vi "LogViewer.vi"(7 "Current Module(\"\" to generate an ID)":string="logViewer") -> ()   [LabVIEW 2017, in "DebugConsole.lvlib"]
uses:
  DebugConsole.lvlib
  Utility/_support/Periodic String Filter Level.ctl
  _BroadcastDef.ctl
  Utility/Periodic String Filter Setting.ctl
  _Shared/Change Speed Counter.vi
  _Shared/Rising Edge.vi
  _Shared/Debounced Signal.vi
  _csmlite/_PassAllowedMessage - MsgList.vi
  Communicable State Machine.lvlib
  _Shared/CSM Shared.lvlib
  _Support/csm-tool-support.lvlib
  _csmHelper/API with lvcsm Support/CSM-Helper API with lvcsm Support.lvlib
  addons/Logger/CSM File Logger.lvlib
  _ui/csm-ui-support.lvlib
  _csmlite/_csmlite.lvlib
panel:
  out "Error(#)":i64 caption="Error(#):"
  in  "Record.Stop":bool
  in  "Record.Start":bool
  in  "Clear":bool
  in  "BackTop":bool
  in  "Toolbar.History Length(char)":i32=50000 caption="History(char)" min=1000 max=100000000 step=1
  in  "Peroid Logs":bool
  in  "Tab":T1(tab)
  out "State History":string
  out "Error History":string
  out "Userlog History":string
  out "Global Filters":string
  out "LogInQ":i32 caption="LogInQ:"
  out "log handling Speed(#/s)":dbl caption="log handling Speed(#/s):"
  out "LogInQ change(#/s)":dbl caption="LogInQ change(#/s):"
  out "Level":T2 caption="Level:"
  in  "Stop":bool
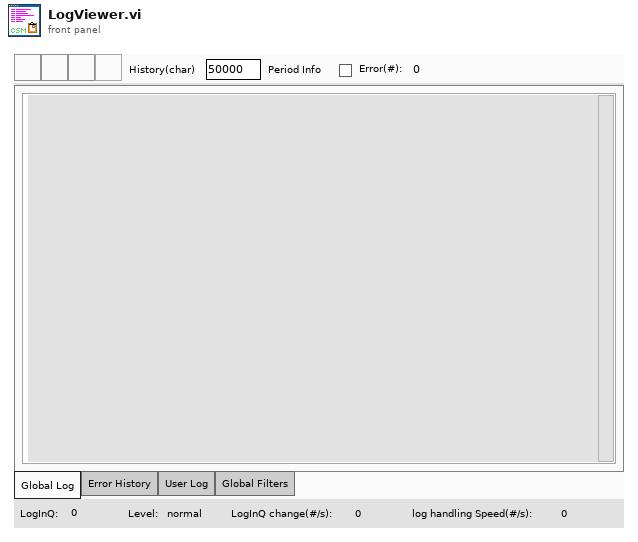
[diagram p1: front panel]
types:
  T1 = enum32{"Global Log", "Error History", "User Log", "Global Filters"}
  T2 = typedef "Communicable State Machine.lvlib/Periodic String Filter Level.ctl" = enum16{"normal", "L1", "L2", "L3", "L4"}
  T3 = typedef "DebugConsole.lvlib/_BroadcastDef.ctl" = enum16{"<no action>", "Macro: Exit", "CSM: Module List Changed", "CSM: Scripts Changed", "CSM: Registration Changed", "CSM: Module Selected", "CSM: Message Excuted", "CSM: Broadcast Excuted", "CSM: Registration Action Excuted", "UI: Try to Change Command"}
  T4 = typedef "Communicable State Machine.lvlib/Periodic String Filter Setting.ctl" = cluster{"threashold(#/s)":dbl, "Check Peroid(s)":dbl}
  T5 = typedef "Communicable State Machine.lvlib/_CSM_GlobalLog_MSG.ctl" = cluster{"Name (\"\" to Use UUID)":string, "Current State":string, "Arguments":string, "Source Message":T6, "Source Module":string, "Complete(T)/Start(F)":bool, "LogType":T7, "Time Stamp":timestamp}
  T6 = typedef "Communicable State Machine.lvlib/_CSM_Response Source Message.ctl" = cluster{"‘State":string, "’Arguments":string, "’Error":errorcluster}
  T7 = typedef "Communicable State Machine.lvlib/_CSM_GlobalLog_MSG_TYPE.ctl" = enum16{"User Log", "State Change", "Status", "Interrupt", "Register", "Unregister", "Error Log", "Module Created", "Module Destroyed", "Async Message", "No-Rep Async Message", "Sync Message"}
  T8 = enum32{"Invalid", "Standard", "Closed", "Hidden", "Minimized", "Maximized"}
  T9 = enum32{"invalid app kind", "Development System", "Run Time System", "Student Edition", "Embedded LabVIEW", "Evaluation", "Custom"}
  T10 = typedef "LVPoint32TypeDef.ctl" = cluster{"Horizontal":i32, "Vertical":i32}
  T11 = cluster{"Shift":bool, "Ctrl":bool, "Alt":bool, "Cmd":bool, "Opt":bool}
  T12 = cluster{"Core":cluster{"Current VI Reference":refnum<vi>, "Close Panel on Exit?":bool}, "Toolbar.Advance":refnum<vi>[], "LoggerWatchDogQueue":refnum<queue>, "LogFile":path}
  T13 = cluster{"Current VI Reference":refnum<vi>, "Close Panel on Exit?":bool}
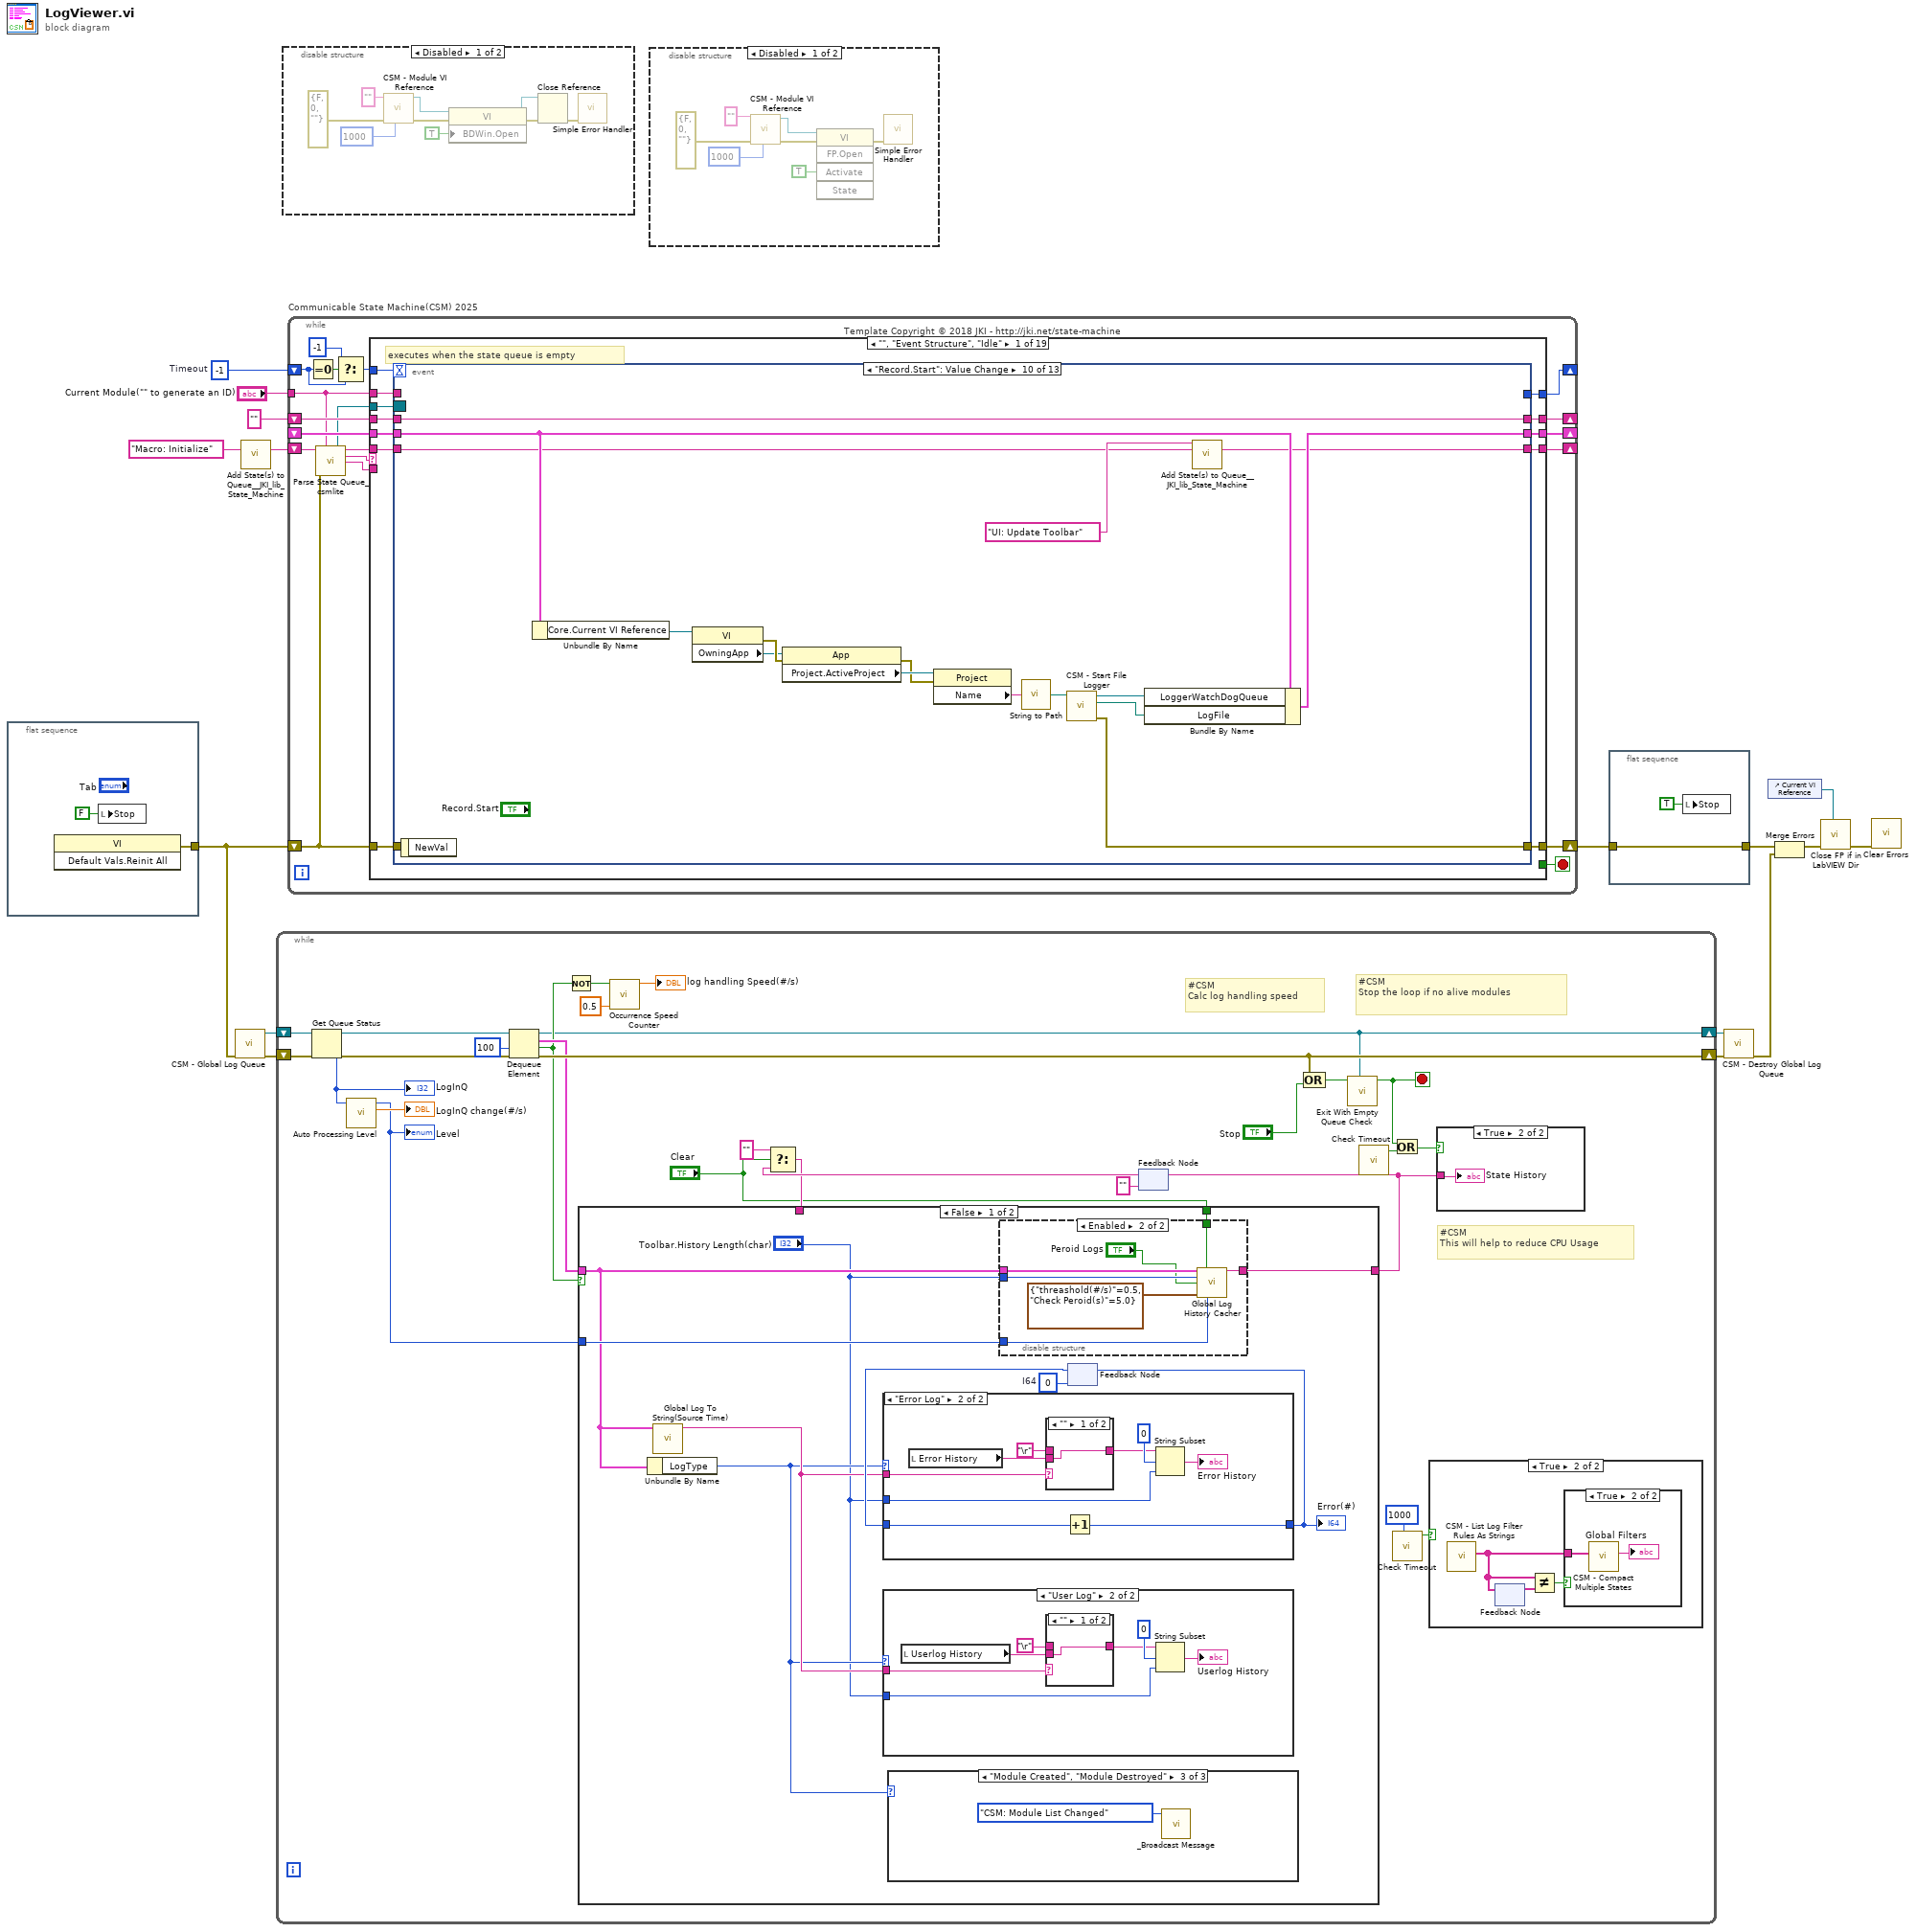
[diagram p0: block diagram]
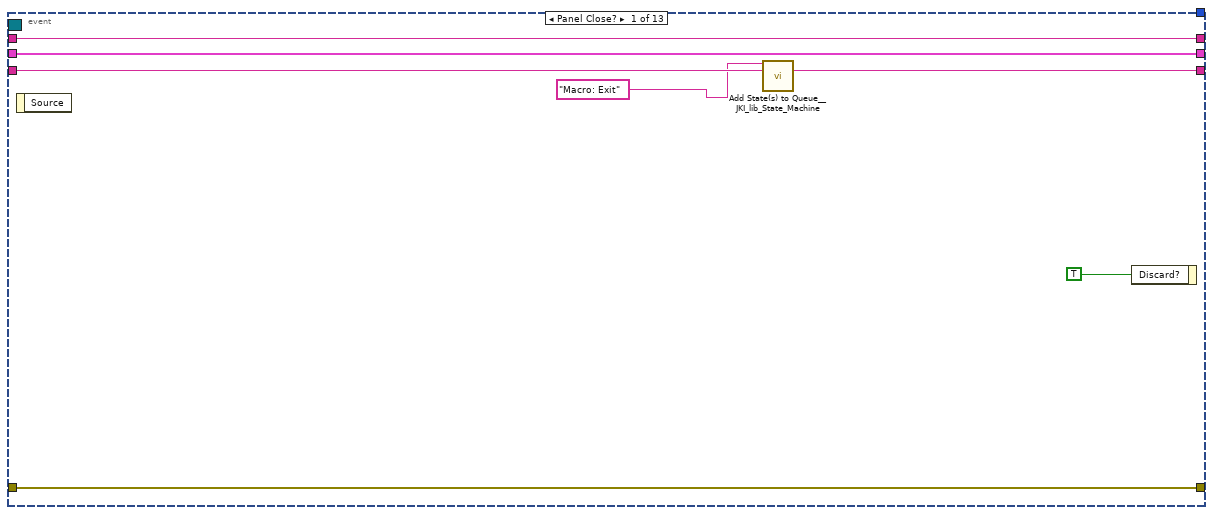
[diagram p4: hidden frame]
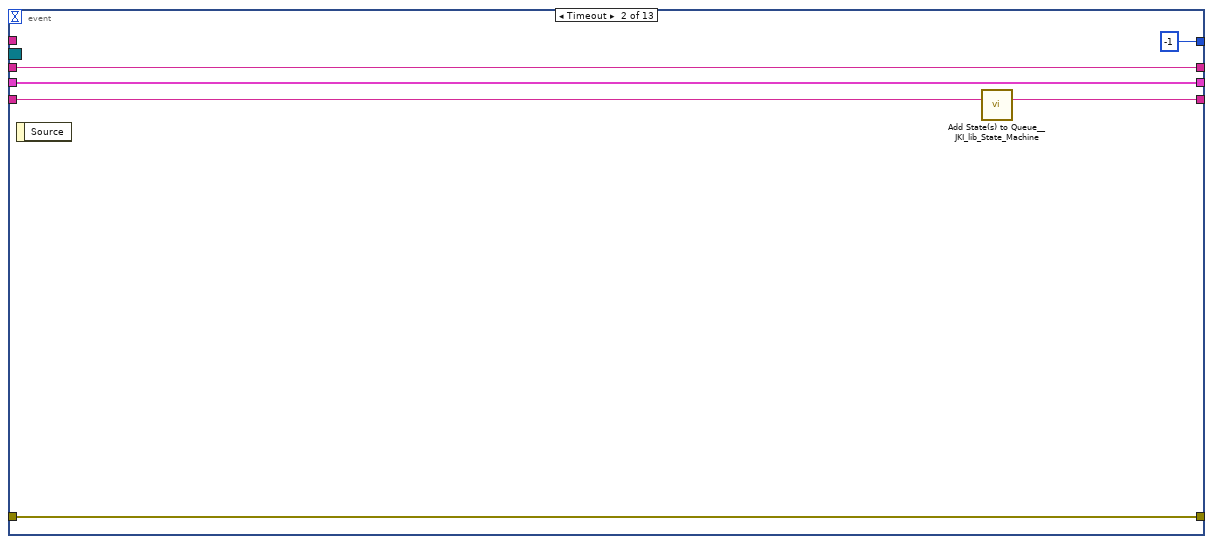
[diagram p5: hidden frame]
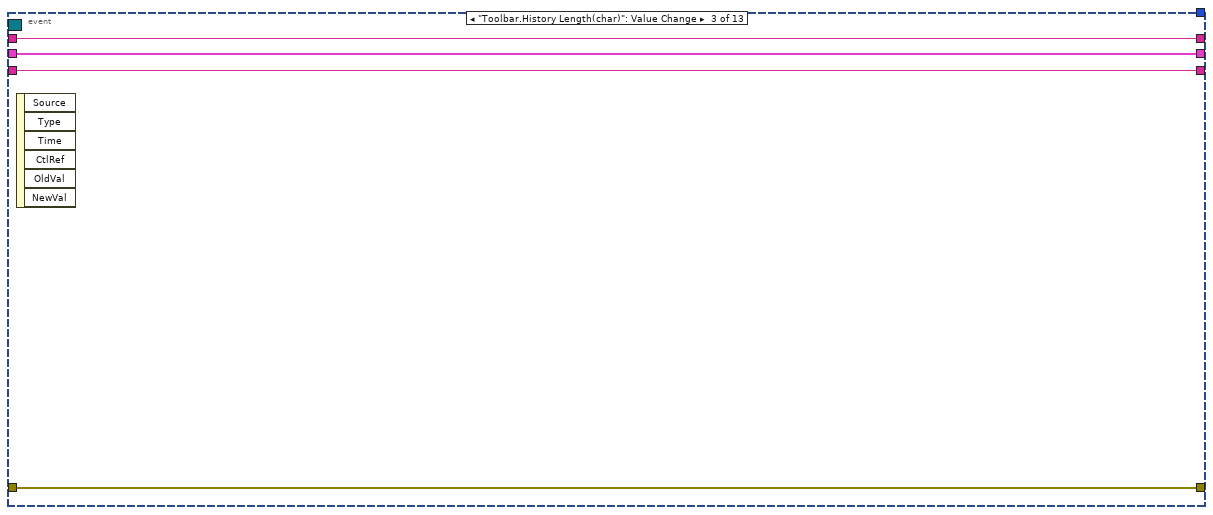
[diagram p6: hidden frame]
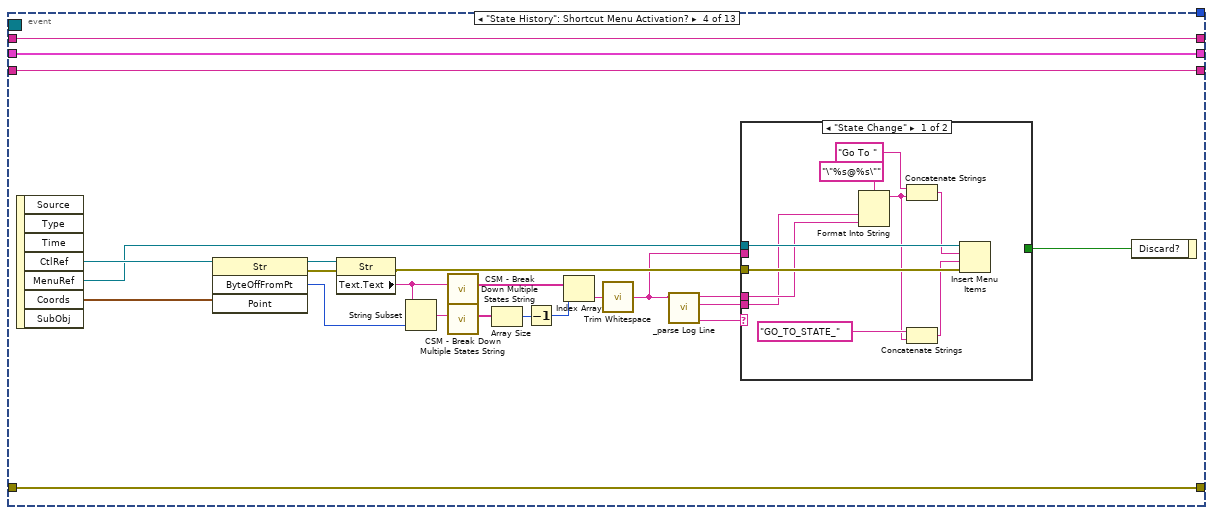
[diagram p7: hidden frame]
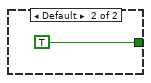
[diagram p8: hidden frame]
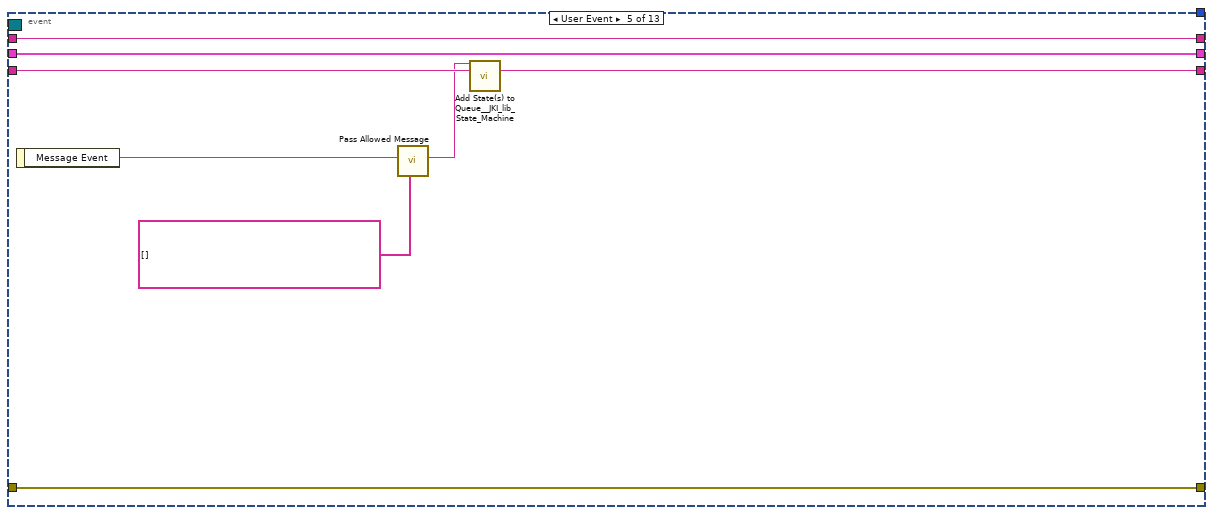
[diagram p9: hidden frame]
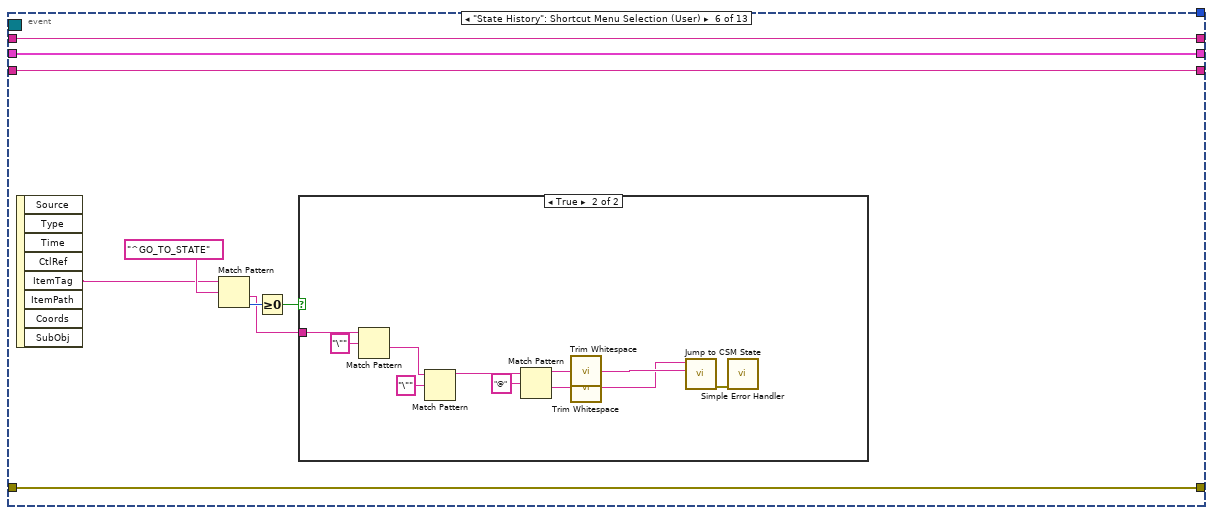
[diagram p10: hidden frame]
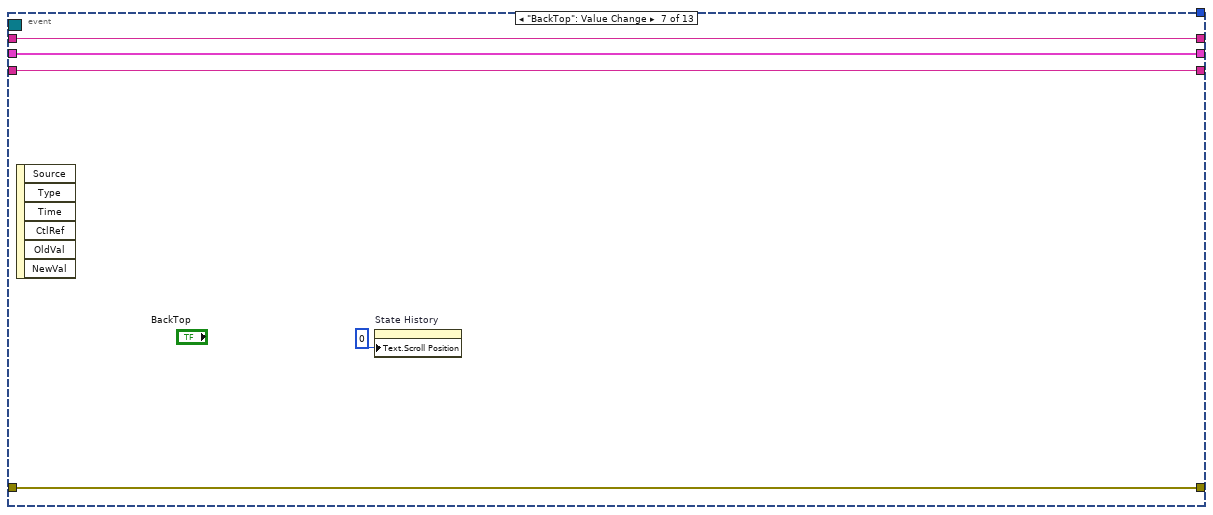
[diagram p12: hidden frame]
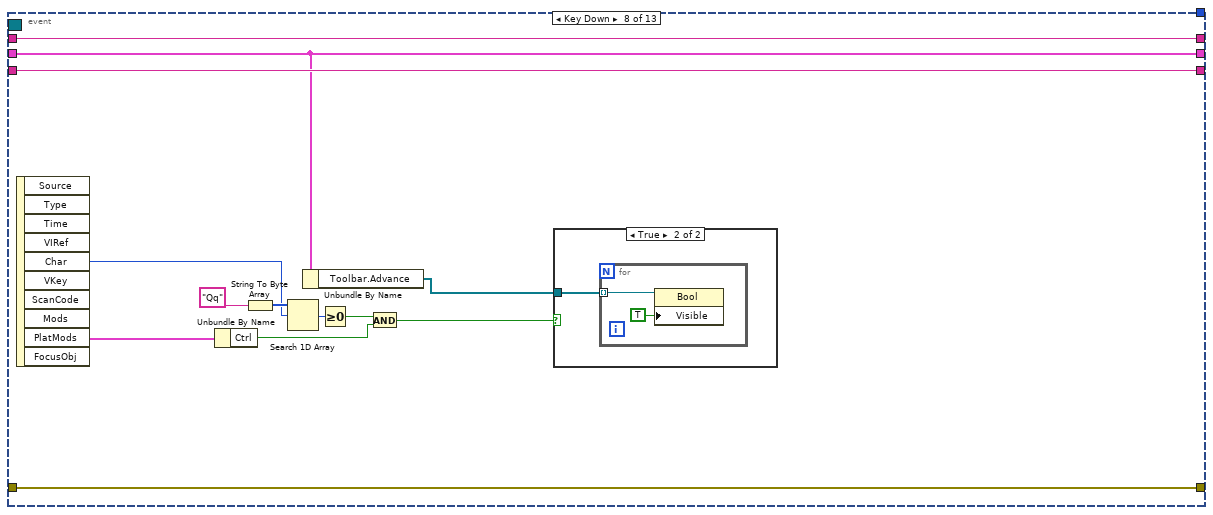
[diagram p13: hidden frame]
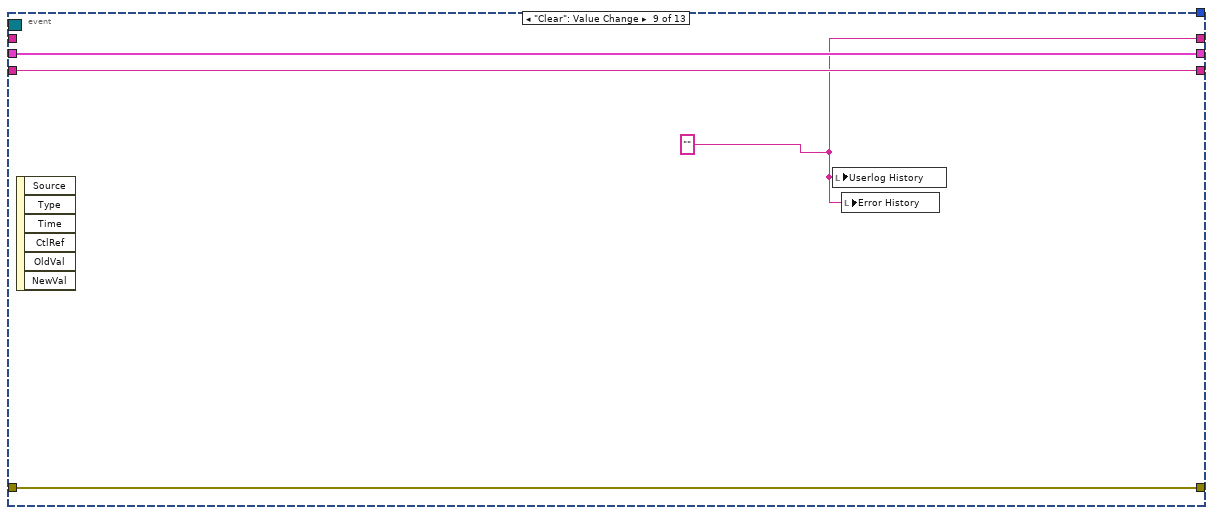
[diagram p15: hidden frame]
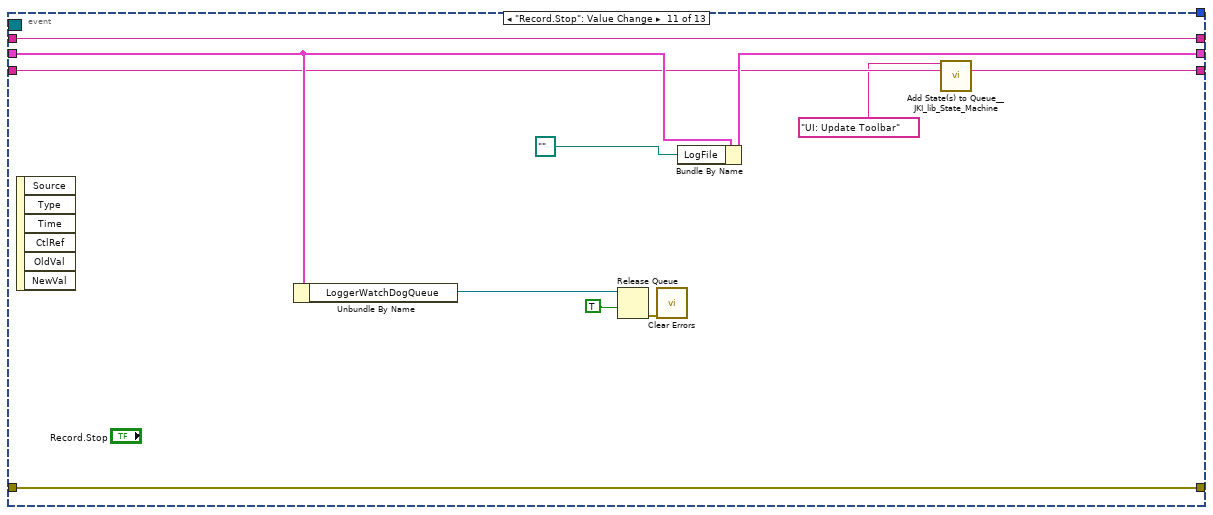
[diagram p16: hidden frame]
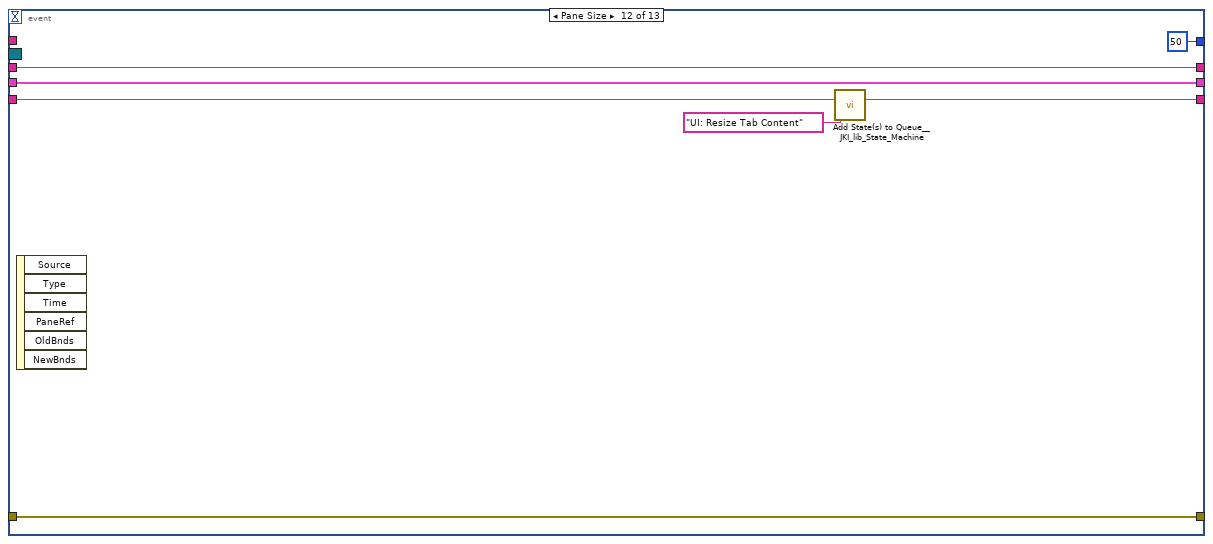
[diagram p17: hidden frame]
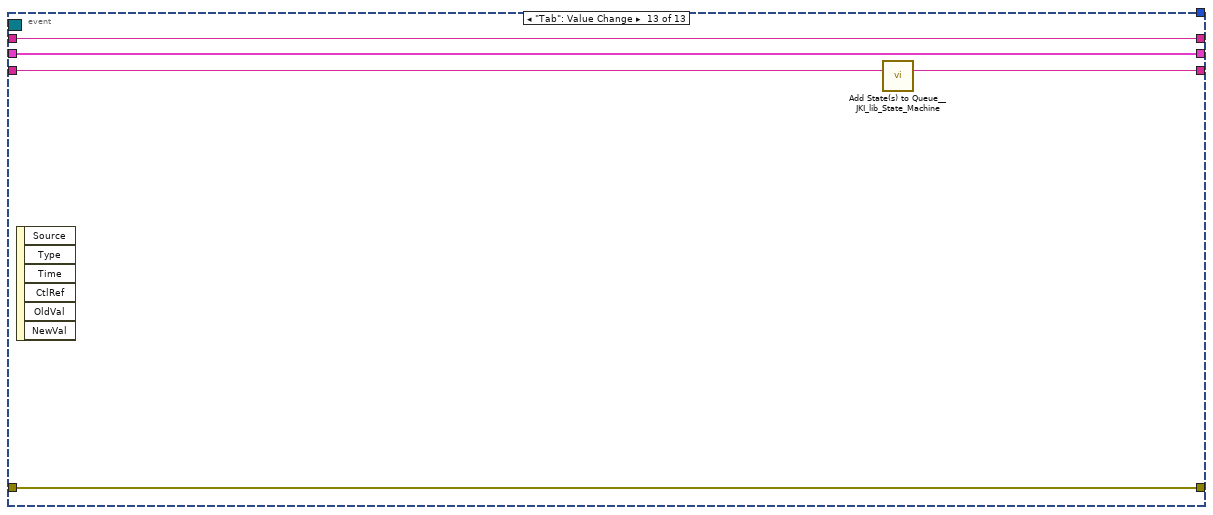
[diagram p18: hidden frame]
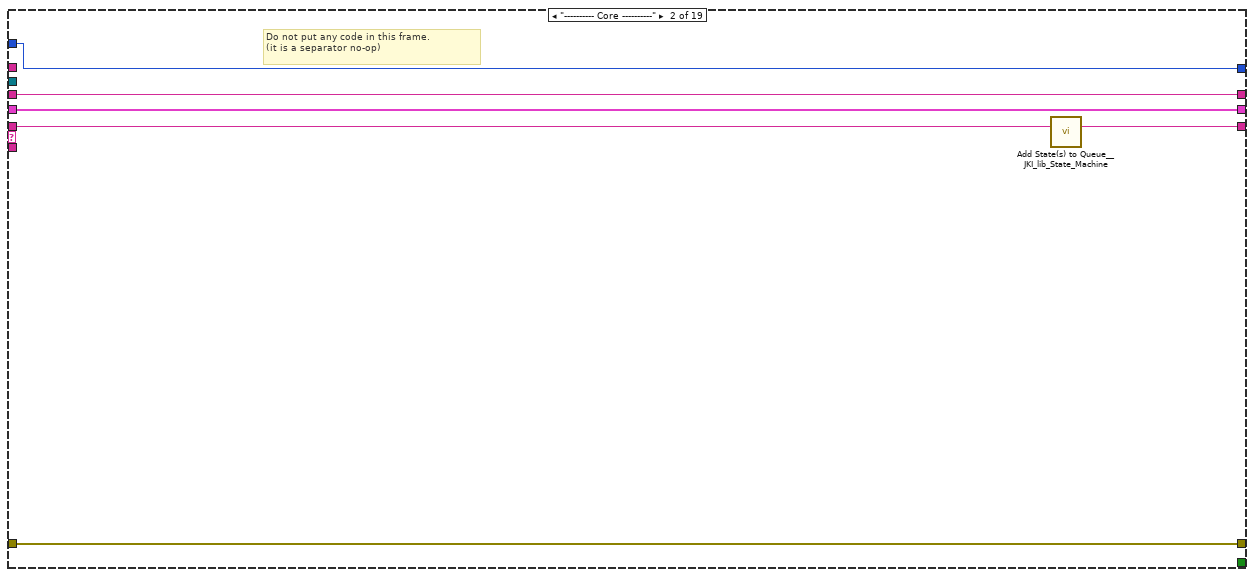
[diagram p19: hidden frame]
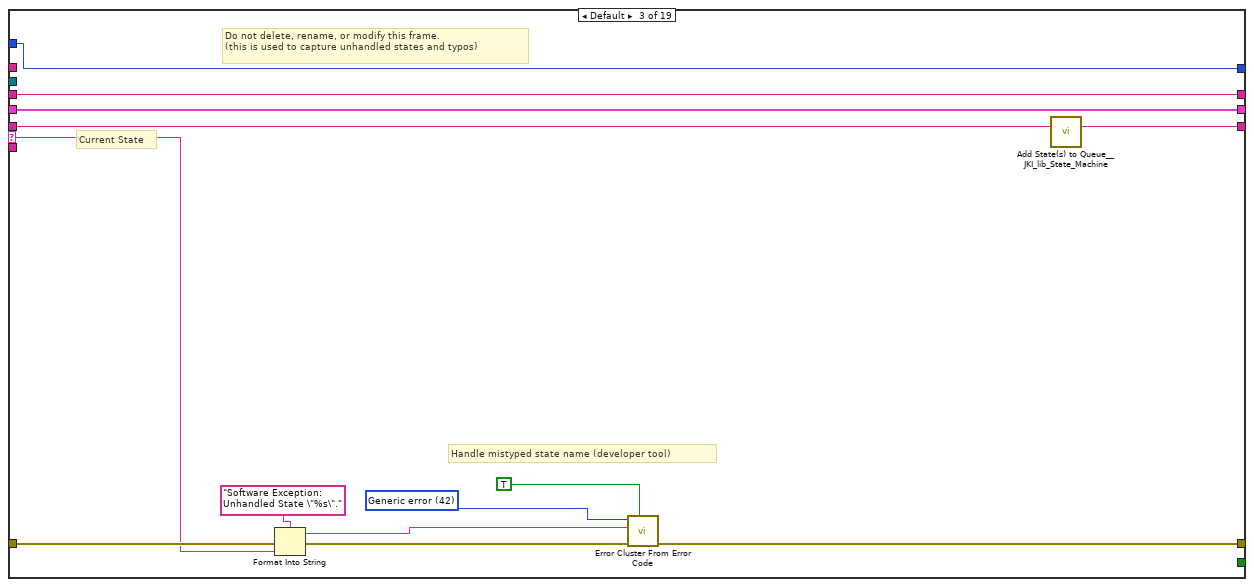
[diagram p20: hidden frame]
diagram:
  w9 = -1  # Timeout
  n1 = flat-sequence {
    tunnel: [w18] -> w1
    frame #0 {
      n2 = invoke class="VI" method="Default Vals.Reinit All"() -> (error out=w18:errorcluster)  [unwired: 3 in, 2 out]
      n3 = local write "Stop"(FALSE ("Stop")) -> ()
    }
  }
  n4 = call "CSM - Global Log Queue.vi"("Error In"=w1) -> ("error out"=w15:errorcluster, "Global Log Queue"=w13:refnum<queue>)  [unwired: 9 in]
  n5 = call <vilib>:"Add State(s) to Queue__JKI_lib_State_Machine.vi"("State(s) in (\"\")"="Macro: Initialize") -> ("States Out"=w12:string)  [unwired: 14 in]
  n6 = while {
    shift-right: [w45] -> w16
    shift-left: w15 -> [w42]
    shift-right: [w33] -> w14
    shift-left: w13 -> [w46]
    stop <- w26 stop-if-true
    # "#CSM\nCalc log handling speed"
    # "#CSM\nStop the loop if no alive modules"
    # "#CSM\nThis will help to reduce CPU Usage"
    n7 = Get Queue Status(queue=w46, error in (no error)=w42) -> (queue out=w44:refnum<queue>, error out=w43:errorcluster, # elements in queue=w29:i32)  [unwired: 1 in, 5 out]
    "LogInQ" <- w29
    n8 = call "Auto Processing Level.vi"("#Left In Q"=w29) -> ("LogInQ Changing Speed (#/s)"=→"LogInQ change(#/s)":dbl, "Level"=w28:T2)  [unwired: 8 in, 1 out]
    "Level" <- w28
    n9 = Dequeue Element(queue=w44, timeout in ms (-1)=100, error in (no error)=w43) -> (queue out=w33:refnum<queue>, element=w41:T5, timed out?=w35:bool, error out=w45:errorcluster)
    n10 = Not(x=w35) -> (.not. x?=w34:bool)
    n11 = call "Occurrence Speed Counter.vi"("Period (0.1s)"=0.5, "Occured? (T)"=w34) -> ("Speed (#/s)"=→"log handling Speed(#/s)":dbl)  [unwired: 7 in, 2 out]
    n12 = feedback #1("" ("String Cache")) -> (w24:string)
    n13 = Select(t="", s="Clear", f=w24) -> (s? t:f=w23:string)
    n14 = case shown="False" w35 {
      tunnel: w41 -> [w59 _]
      tunnel: [w61 w101] -> w38
      tunnel: w23 -> [_ w101]
      tunnel: w28 -> [w60 _]
      tunnel: "Clear" -> [w52 _]
      frame False {
        w57 = i64 0  # I64
        n15 = Unbundle By Name(w59) -> ("LogType"=w54:T7)
        n16 = call "Global Log To String(Source Time).vi"("Log"=w59) -> ("Log String"=w55:string)  [unwired: 9 in]
        n17 = case shown="\"User Log\"" w54 {
          tunnel: w55 -> [_ w63]
          tunnel: "Toolbar.History Length(char)" -> [_ w62]
          frame Default {
          }
          frame "User Log" {
            n18 = local read "Userlog History"() -> (w67:string)
            n19 = case shown="\"\"" w63 {
              selector: w63 -> [_ w70]
              tunnel: "\r" -> [_ w73]
              tunnel: w67 -> [w69 w72]
              tunnel: [w69 w71] -> w65
              frame "" {
              }
              frame Default {
                n20 = Concatenate Strings(w70, w73, w72) -> (w71:string)
              }
            }
            n21 = String Subset(string=w65, offset (0)=0, length (rest)=w62) -> (substring=→"Userlog History":string)
          }
        }
        n22 = case shown="\"Module Created\", \"Module Destroyed\"" w54 {
          frame "User Log", Default {
          }
          frame "Register", "Unregister" {
            n23 = call "_Broadcast Message.vi"("Broadcast"=_BroadcastDef."CSM: Registration Changed") -> ()  [unwired: 10 in, 1 out]
          }
          frame "Module Created", "Module Destroyed" {
            n24 = call "_Broadcast Message.vi"("Broadcast"=_BroadcastDef."CSM: Module List Changed") -> ()  [unwired: 10 in, 1 out]
          }
        }
        n25 = disable-structure shown="Enabled" {
          disable-tunnel: w59 -> [w93 w99]
          disable-tunnel: [w91 w100] -> w61
          disable-tunnel: w60 -> [_ w98]
          disable-tunnel: "Toolbar.History Length(char)" -> [_ w96]
          disable-tunnel: w52 -> [_ w94]
          frame Disabled {
            # "#CSM \nno periodical filter"
            n26 = call "Global Log To String(Source Time).vi"("Log"=w93) -> ("Log String"=w92:string)  [unwired: 9 in]
            n27 = call "String History Cacher.vi"("String"=w92) -> ("String Cache"=w91:string)  [unwired: 10 in]
          }
          frame Enabled {
            n28 = call "Global Log History Cacher.vi"("Global Log Data"=w99, "Reset?"=w94, "Length (10000)"=w96, "With Periodic Info? (T)"="Peroid Logs", "Settings"=T4 {"threashold(#/s)"=0.5, "Check Peroid(s)"=5.0}, "Level (Normal)"=w98) -> ("String Cache"=w100:string)  [unwired: 9 in]
          }
        }
        n29 = feedback #2(w57) -> (w56:i64)
        n30 = case shown="\"Error Log\"" w54 {
          tunnel: w55 -> [_ w80]
          tunnel: "Toolbar.History Length(char)" -> [_ w79]
          tunnel: [w76 w78] -> w58
          tunnel: w56 -> [w76 w77]
          frame "User Log", Default {
          }
          frame "Error Log" {
            n31 = local read "Error History"() -> (w84:string)
            n32 = case shown="\"\"" w80 {
              selector: w80 -> [_ w87]
              tunnel: "\r" -> [_ w90]
              tunnel: w84 -> [w86 w89]
              tunnel: [w86 w88] -> w82
              frame "" {
              }
              frame Default {
                n33 = Concatenate Strings(w87, w90, w89) -> (w88:string)
              }
            }
            n34 = Increment(x=w77) -> (x+1=w78:i64)
            n35 = String Subset(string=w82, offset (0)=0, length (rest)=w79) -> (substring=→"Error History":string)
          }
        }
        "Error(#)" <- w58
        n36 = feedback-in #2(w58) -> ()
      }
      frame True {
      }
    }
    n37 = feedback-in #1(w38) -> ()
    n38 = Compound Arithmetic op=OR(w45, "Stop") -> (w31:bool)
    n39 = call "Exit With Empty Queue Check.vi"("Queue"=w33, "Stop"=w31) -> ("Exit"=w26:bool)  [unwired: 8 in, 1 out]
    n40 = call "Check Timeout.vi"() -> ("Timeout"=w39:bool)  [unwired: 8 in]
    n41 = Or(x=w26, y=w39) -> (x .or. y?=w32:bool)
    n42 = call "Check Timeout.vi"("Timeout Expected (ms)"=1000) -> ("Timeout"=w20:bool)  [unwired: 7 in]
    n43 = case shown="True" w20 {
      frame False {
      }
      frame True {
        n44 = call "CSM - List Log Filter Rules As Strings.vi"() -> ("Rule Strings"=w47:string[])  [unwired: 10 in, 1 out]
        n45 = feedback-in #3(w47) -> ()
        n46 = feedback #3() -> (w48:string[])  [unwired: 1 in]
        n47 = Not Equal?(x=w47, y=w48) -> (x != y?=w49:bool)
        n48 = case shown="True" w49 {
          tunnel: w47 -> [_ w50]
          frame False {
          }
          frame True {
            n49 = call "CSM - Compact Multiple States.vi"("Multiple States"=w50) -> ("States"=→"Global Filters":string)  [unwired: 9 in]
          }
        }
      }
    }
    n50 = case shown="True" w32 {
      tunnel: w38 -> [_ w102]
      frame False {
      }
      frame True {
        "State History" <- w102
      }
    }
  }
  n51 = disable-structure shown="Disabled" {
    frame Disabled {
      n52 = call "CSM - Module VI Reference.vi"("Response Timeout (-2 Using Global Settings)"=1000 ("Response Timeout(5000 ms)"), "error in (no error)"=errorcluster {"status"=FALSE, "code"=0, "source"=""}, "CSM Name"="") -> ("error out"=w111:errorcluster, "CSM Module VIRef"=w108:refnum<vi>)  [unwired: 7 in]
      n53 = property class="VI"(reference=w108, error in=w111, "BDWin.Open"=TRUE ("Block Diagram Window:Open")) -> (reference out=w109:refnum<vi>, error out=w110:errorcluster)
      n54 = Close Reference(reference=w109, error in (no error)=w110) -> (error out=w107:errorcluster)
      n55 = call <vilib>:"Simple Error Handler.vi"("error in (no error)"=w107) -> ()  [unwired: 4 in, 5 out]
    }
    frame Enabled {
    }
  }
  n56 = while "Communicable State Machine(CSM) 2025" {
    shift-right: [w123] -> _
    shift-left: _ -> [w122]
    shift-right: [w126] -> w6
    shift-left: w1 -> [w121]
    shift-right: [w125] -> _
    shift-left: w12 -> [w127]
    tunnel: "Current Module(\"\" to generate an ID)" -> [w113]
    shift-right: [w119] -> _
    shift-left: "" ("String Cache") -> [w120]
    shift-right: [w118] -> _
    shift-left: w9 -> [w115]
    stop <- w124 stop-if-true
    # "Template Copyright © 2018 JKI - http://jki.net/state-machine"
    n57 = Equal To 0?(x=w115) -> (x = 0?=w117:bool)
    n58 = call "Parse State Queue_csmlite.vi"("State Queue"=w127, "Current Module(\"\" to generate an ID)"=w113, "Error In (no error)"=w121) -> ("Event Registration Refnum"=w112:refnum<event-registration>, "Remaining States"=w129:string, "Current State"=w130:string, "Arguments"=w128:string)  [unwired: 9 in]
    n59 = Select(t=-1 ("Timeout"), s=w117, f=w115) -> (s? t:f=w116:i32)
    n60 = case shown="\"\", \"Event Structure\", \"Idle\"" w130 {
      selector: w130 -> [_ _ w294 _ _ _ _ _ _ _ _ _ _ _ _ _ _ _ _]
      tunnel: w129 -> [w142 w291 w298 w319 w327 w334 w340 w350 w355 w363 w369 w387 w398 w411 w495 w514 w524 w531 w539]
      tunnel: w128 -> [_ _ _ _ _ _ _ _ _ _ _ _ w393 w405 _ _ _ _ _]
      tunnel: w122 -> [w140 w288 w296 w312 w324 w332 w337 _ w354 w358 w366 w383 w396 w407 w491 w513 w521 w528 w536]
      tunnel: [w139 w289 w300 w316 errorcluster {"status"=FALSE, "code"=0, "source"=""} ("error out") w331 w338 w347 w352 w359 w367 w385 w394 w408 w496 w515 w522 w529 w537] -> w126
      tunnel: w121 -> [w138 w289 w299 w316 w323 w331 w338 w347 w352 w360 w367 w385 w395 w409 w496 w515 w522 w529 w537]
      tunnel: [w141 w290 w297 w318 w326 w333 w339 w349 w355 w362 w368 w386 w397 w410 w495 w514 w523 w530 w538] -> w125
      tunnel: [_ _ _ _ _ TRUE _ _ _ _ _ _ _ _ _ _ _ _ _] -> w124
      tunnel: [w137 w288 w296 w317 w324 w332 w337 w348 w354 w358 w366 w383 w396 w407 w491 w513 w521 w528 w536] -> w123
      tunnel: w116 -> [w136 w286 w292 w305 w320 w328 w335 w341 w351 w356 w364 w380 w391 w403 w477 w511 w519 w525 w532]
      tunnel: w112 -> [w135 _ _ _ _ _ _ _ _ _ _ _ _ _ _ _ _ _ _]
      tunnel: w113 -> [w134 _ _ _ _ _ _ _ _ _ _ _ _ _ _ _ _ _ _]
      tunnel: w120 -> [w133 w287 w293 w306 w321 w329 w336 w345 w353 w357 w365 w384 w392 w404 w494 w512 w520 w526 w533]
      tunnel: [w132 w287 w293 w306 w321 w329 w336 w345 w353 w357 w365 w384 w392 w404 w494 w512 w520 w526 w533] -> w119
      tunnel: [w131 w286 w292 w305 w320 w328 w335 w341 w351 w356 w364 w380 w391 w403 w477 w511 w519 w525 w532] -> w118
      frame "", "Event Structure", "Idle" {
        # "executes when the state queue is empty"
        n61 = event shown="[9] \"Record.Start\": Value Change" {
          selector: w135 -> [_ _ _ _ _ _ _ _ _ _ _ _ _]
          dyn-events: _ -> [_ _ _ _ _ _ _ _ _ _ _ _ _]
          timeout: w136 -> [_ _ _ _ _ _ _ _ _ _ _ _ _]
          tunnel: w142 -> [w149 w155 w159 w182 w197 w210 w226 w239 w246 w248 w265 w276 w281]
          tunnel: [w148 w154 w159 w182 w198 w210 w226 w239 w246 w247 w264 w277 w282] -> w141
          tunnel: w140 -> [w146 w152 w157 w180 w200 w208 w224 w229 w244 w257 w271 w279 w284]
          tunnel: [w147 w153 w158 w181 w201 w209 w225 w238 w245 w259 w273 w280 w285] -> w139
          tunnel: w138 -> [w147 w153 w158 w181 w201 w209 w225 w238 w245 _ w273 w280 w285]
          tunnel: [w146 w152 w157 w180 w200 w208 w224 w229 w244 w260 w267 w279 w284] -> w137
          tunnel: w134 -> [_ _ _ _ _ _ _ _ _ _ _ _ _]
          tunnel: w133 -> [w143 w151 w156 w179 w199 w207 w223 w237 _ w262 w272 w278 w283]
          tunnel: [w143 w151 w156 w179 w199 w207 w223 w237 w243 w262 w272 w278 w283] -> w132
          tunnel: [_ -1 ("Timeout") _ _ _ _ _ _ _ _ _ 50 ("Timeout") _] -> w131
          event Panel Close? {
            n62 = event-data() -> ()  [unwired: 1 in, 1 out]
            n63 = call <vilib>:"Add State(s) to Queue__JKI_lib_State_Machine.vi"("State(s) in Front (\"\")"="Macro: Exit", "State(s) in (\"\")"=w149) -> ("States Out"=w148:string)  [unwired: 13 in]
            n64 = event-data("Discard?"=TRUE) -> ()  [unwired: 1 in, 1 out]
          }
          event Timeout {
            n65 = event-data() -> ()  [unwired: 1 in, 1 out]
            n66 = call <vilib>:"Add State(s) to Queue__JKI_lib_State_Machine.vi"("State(s) in (\"\")"=w155) -> ("States Out"=w154:string)  [unwired: 14 in]
          }
          event "Toolbar.History Length(char)": Value Change {
            n67 = event-data() -> ()  [unwired: 1 in, 6 out]
          }
          event "State History": Shortcut Menu Activation? {
            n68 = event-data() -> ("CtlRef"=w162:refnum<vi>, "MenuRef"=w161:refnum<k9>, "Coords"=w160:T10)  [unwired: 1 in, 4 out]
            n69 = invoke class="Str" method="ByteOffFromPt"(reference=w162, "Point"=w160) -> (reference out=w178:refnum<vi>, error out=w176:errorcluster, "ByteOffFromPt"=w177:i32)  [unwired: 2 in, 1 out]
            n70 = property class="Str"(reference=w178, error in=w176) -> (error out=w168:errorcluster, "Text.Text"=w174:string)  [unwired: 1 out]
            n71 = String Subset(string=w174, length (rest)=w177) -> (substring=w175:string)  [unwired: 1 in]
            n72 = call "CSM - Break Down Multiple States String.vi"("States"=w174) -> ("Multiple States"=w173:string[])  [unwired: 10 in]
            n73 = call "CSM - Break Down Multiple States String.vi"("States"=w175) -> ("Multiple States"=w172:string[])  [unwired: 10 in]
            n74 = Array Size(array=w172) -> (size(s)=w171:i32)
            n75 = Decrement(x=w171) -> (x-1=w170:i32)
            n76 = Index Array(array=w173, index=w170) -> (element=w169:string)
            n77 = call <vilib>:"Trim Whitespace.vi"("string"=w169) -> ("trimmed string"=w167:string)  [unwired: 1 in]
            n78 = call "_parse Log Line.vi"("String"=w167) -> ("LogType"=w166:string, "State"=w164:string, "CSM"=w165:string)  [unwired: 8 in]
            n79 = case shown="\"State Change\"" w166 {
              tunnel: w161 -> [w192 _]
              tunnel: w167 -> [_ _]
              tunnel: w168 -> [w190 _]
              tunnel: [_ TRUE] -> w163
              tunnel: w165 -> [w188 _]
              tunnel: w164 -> [w187 _]
              frame "State Change" {
                n80 = Format Into String(format string="\"%s@%s\"", w187, w188) -> (resulting string=w183:string)  [unwired: 2 in, 1 out]
                n81 = Concatenate Strings("Go To " ("format string"), w183) -> (w186:string)
                n82 = Concatenate Strings("GO_TO_STATE_" ("item tags"), w183) -> (w184:string)
                n83 = Insert Menu Items(6:w190, 7:w184, 8:w186, 9:w192) -> ()  [unwired: 2 in, 3 out]
              }
              frame Default {
              }
            }
            n84 = event-data("Discard?"=w163) -> ()  [unwired: 1 in, 1 out]
          }
          event User Event {
            n85 = event-data() -> ("Message Event"=w195:string)  [unwired: 1 in]
            n86 = call-poly "Pass Allowed Message.vi"("Allowed Message"=string[] [] ("1D array"), "JKISM External Event"=w195) -> ("States"=w196:string)  [unwired: 7 in]
            n87 = call <vilib>:"Add State(s) to Queue__JKI_lib_State_Machine.vi"("State(s) in Front (\"\")"=w196, "State(s) in (\"\")"=w197) -> ("States Out"=w198:string)  [unwired: 13 in]
          }
          event "State History": Shortcut Menu Selection (User) {
            n88 = event-data() -> ("ItemTag"=w202:string)  [unwired: 1 in, 7 out]
            n89 = Match Pattern(string=w202, regular expression="^GO_TO_STATE") -> (after substring=w203:string, offset past match=w205:i32)  [unwired: 1 in, 2 out]
            n90 = Greater Or Equal To 0?(x=w205) -> (x >= 0?=w204:bool)
            n91 = case shown="True" w204 {
              tunnel: w203 -> [_ w221]
              frame False {
              }
              frame True {
                n92 = Match Pattern(string=w221, regular expression="\"") -> (after substring=w218:string)  [unwired: 1 in, 3 out]
                n93 = Match Pattern(string=w218, regular expression="\"") -> (before substring=w217:string)  [unwired: 1 in, 3 out]
                n94 = Match Pattern(string=w217, regular expression="@") -> (before substring=w215:string, after substring=w214:string)  [unwired: 1 in, 2 out]
                n95 = call <vilib>:"Trim Whitespace.vi"("string"=w215) -> ("trimmed string"=w213:string)  [unwired: 1 in]
                n96 = call <vilib>:"Trim Whitespace.vi"("string"=w214) -> ("trimmed string"=w212:string)  [unwired: 1 in]
                n97 = call "Jump to CSM State.vi"("State"=w213, "Name"=w212) -> ("error out"=w211:errorcluster)  [unwired: 9 in]
                n98 = call <vilib>:"Simple Error Handler.vi"("error in (no error)"=w211) -> ()  [unwired: 4 in, 5 out]
              }
            }
          }
          event "BackTop": Value Change {
            n99 = event-data() -> ()  [unwired: 1 in, 6 out]
            n100 = property on="State History" class="Str"("Text.Scroll Position"=u32 0) -> ()  [unwired: 2 in, 2 out]
          }
          event Key Down {
            n101 = event-data() -> ("Char"=w227:i16, "PlatMods"=w232:T11)  [unwired: 1 in, 8 out]
            n102 = Unbundle By Name(w232) -> ("Ctrl"=w231:bool)
            n103 = String To Byte Array(string="Qq") -> (unsigned byte array=w234:u8[])
            n104 = Search 1D Array(1D array=w234, element=w227) -> (index of element=w235:i32)  [unwired: 1 in]
            n105 = Unbundle By Name(w229) -> ("Toolbar.Advance"=w228:refnum<vi>[])
            n106 = Greater Or Equal To 0?(x=w235) -> (x >= 0?=w236:bool)
            n107 = And(x=w236, y=w231) -> (x .and. y?=w230:bool)
            n108 = case shown="True" w230 {
              tunnel: w228 -> [_ w240]
              frame False {
              }
              frame True {
                n109 = for {
                  tunnel: w240 -> [w242] mode=indexing
                  n110 = property class="Bool"(reference=w242, "Visible"=TRUE) -> ()  [unwired: 1 in, 2 out]
                }
              }
            }
          }
          event "Clear": Value Change {
            w243 = "" ("String Cache")
            n111 = event-data() -> ()  [unwired: 1 in, 6 out]
            n112 = local write "Userlog History"(w243) -> ()
            n113 = local write "Error History"(w243) -> ()
          }
          event "Record.Start": Value Change {
            n114 = event-data() -> ()  [unwired: 1 in, 1 out]
            n115 = Unbundle By Name(w257) -> ("Core.Current VI Reference"=w256:refnum<vi>)
            n116 = property class="VI"(reference=w256) -> (error out=w255:errorcluster, "OwningApp"=w254:refnum<vi>)  [unwired: 1 in, 1 out]
            n117 = property class="App"(reference=w254, error in=w255) -> (error out=w252:errorcluster, "Project.ActiveProject"=w253:refnum<vi>)  [unwired: 1 out]
            n118 = property class="Project"(reference=w253, error in=w252) -> ("Name"=w251:string)  [unwired: 2 out]
            n119 = call "String to Path.vi"("String"=w251) -> ("Path"=w250:path)
            n120 = call "CSM - Start File Logger.vi"("Log File Path"=w250) -> ("error out"=w259:errorcluster, "Log File"=w258:path, "Watchdog Queue"=w261:refnum<queue>)  [unwired: 8 in]
            n121 = Bundle By Name(cluster=w257, "LoggerWatchDogQueue"=w261, "LogFile"=w258) -> (w260:T12)
            n122 = call <vilib>:"Add State(s) to Queue__JKI_lib_State_Machine.vi"("State(s) in Front (\"\")"="UI: Update Toolbar" ("State(s) in Front (\"\")"), "State(s) in (\"\")"=w248) -> ("States Out"=w247:string)  [unwired: 13 in]
          }
          event "Record.Stop": Value Change {
            n123 = event-data() -> ()  [unwired: 1 in, 6 out]
            n124 = Unbundle By Name(w271) -> ("LoggerWatchDogQueue"=w270:refnum<queue>)
            n125 = Release Queue(queue=w270, force destroy? (F)=TRUE) -> (error out=w268:errorcluster)  [unwired: 1 in, 2 out]
            n126 = call <vilib>:"Clear Errors.vi"("error in (no error)"=w268) -> ()  [unwired: 5 in, 2 out]
            n127 = Bundle By Name(cluster=w271, "LogFile"=path "") -> (w267:T12)
            n128 = call <vilib>:"Add State(s) to Queue__JKI_lib_State_Machine.vi"("State(s) in Front (\"\")"="UI: Update Toolbar" ("State(s) in Front (\"\")"), "State(s) in (\"\")"=w265) -> ("States Out"=w264:string)  [unwired: 13 in]
          }
          event Pane Size {
            n129 = event-data() -> ()  [unwired: 1 in, 6 out]
            n130 = call <vilib>:"Add State(s) to Queue__JKI_lib_State_Machine.vi"("State(s) in (\"\")"=w276, "State(s) at Back (\"\")"="UI: Resize Tab Content" ("State(s) in Front (\"\")")) -> ("States Out"=w277:string)  [unwired: 13 in]
          }
          event "Tab": Value Change {
            n131 = event-data() -> ()  [unwired: 1 in, 6 out]
            n132 = call <vilib>:"Add State(s) to Queue__JKI_lib_State_Machine.vi"("State(s) in (\"\")"=w281) -> ("States Out"=w282:string)  [unwired: 14 in]
          }
        }
      }
      frame "---------- Core ----------" {
        # "Do not put any code in this frame.\n(it is a separator no-op)"
        n133 = call <vilib>:"Add State(s) to Queue__JKI_lib_State_Machine.vi"("State(s) in (\"\")"=w291) -> ("States Out"=w290:string)  [unwired: 14 in]
      }
      frame Default {
        w303 = 42 items=["No error", "Argument error", "Memory is full", "Out of zone", "End of file", "File already open", "Generic file I/O error", "File not found", "File permission error", "Disk is full", "Duplicate path", "Too many files open", "System feature not enabled", "Resource file not found", "Cannot add resource", "Resource not found", "Image not found", "Image memory error", "Pen does not exist", "Config type invalid", "Config token not found", "Config parse error", "Config memory error", "Bad external code format", "Bad external code offset", "External code not present", "Null window", "Destroy window error", "Null menu", "Print aborted", "Bad print record", "Print driver error", "Windows error during printing", "Memory error during printing", "Print dialog error", "Generic print error", "Invalid device refnum", "Device not found", "Device parameter error", "Device unit error", "Cannot open device", "Device call aborted", "Generic error", "Cancelled by user", "Object ID too low", "Object ID too high", "Object not in heap", "Unknown heap", "Unknown object (invalid DefProc)", "Unknown object (DefProc not in table)", "Message out of range", "Invalid (null) method", "Unknown message", "Manager call not supported", "Bad address", "Network operation in progress", "Network operation timed out", "Connection is busy", "Network attribute not supported", "Network error", "Address in use", "System out of memory", "Connection aborted", "Connection refused", "Not connected", "Already connected", "Connection closed", "Initialization error (interapplication manager)", "Bad occurrence", "Wait on unbound occurrence handler", "Occurrence queue overflow", "Datalog type conflict", "Unused", "Unrecognized type (interapplication manager)", "Memory corrupt", "Failed to make temporary DLL", "Old CIN version", "Drag socket not found", "Failed to load drop-object", "Failed to register OLE object", "Failed to release OLE object", "Format specifier type mismatch", "Unknown format specifier", "Too few format specifiers", "Too many format specifiers", "Scan failed", "Newer CIN version", "Error converting to variant", "Runtime menu error", "Password tampered", "Variant attribute not found", "Incompatible variant data type", "Event data is not available", "Event Store is not present", "Occurrence is not found", "Event Queue is not created", "Event info is not available", "Refnum passed is NULL", "Error retrieving Class GUID", "Error retrieving CoClass GUID", "Error retrieving TypeLib GUID.", "Bad built application magic bytes.", "Specific driver is different from the specific driver associated with the Logical Name.", "There is no session opened to the class driver.", "Max Error", "MAX - Error with config objects", "MAX - Error loading configuration", "MAX - Group not supported"]
        # "Current State"
        # "Do not delete, rename, or modify this frame.\n(this is used to capture unhandled states and typos)"
        # "Handle mistyped state name (developer tool)"
        n134 = Format Into String(format string="Software Exception: Unhandled State \"%s\"." ("message"), error in=w299, w294) -> (resulting string=w302:string, error out=w301:errorcluster)  [unwired: 1 in]
        n135 = call <vilib>:"Error Cluster From Error Code.vi"("show call chain? (False)"=TRUE, "error in (no error)"=w301, "error message (\"\")"=w302, "error code (0)"=w303) -> ("error out"=w300:errorcluster)  [unwired: 5 in]
        n136 = call <vilib>:"Add State(s) to Queue__JKI_lib_State_Machine.vi"("State(s) in (\"\")"=w298) -> ("States Out"=w297:string)  [unwired: 14 in]
      }
      frame "Initialize Core Data" {
        # "Do not delete, rename, or modify this frame.\n(this is used to determine panel behavior on exit)"
        # "originally closed?"
        # "exe?"
        # "If panel starts closed or is an EXE, then close it when we exit"
        n137 = property class="VI"() -> ("FP.State"=w309:T8)  [unwired: 2 in, 2 out]
        n138 = property class="App"() -> ("App.Kind"=w315:T9)  [unwired: 2 in, 2 out]
        n139 = control-ref of="Current VI Reference"() -> (w310:refnum<vi>)
        n140 = Equal?(x=w309, y=T8."Closed" ("Front Panel Window:State")) -> (x = y?=w307:bool)
        n141 = Equal?(x=w315, y=T9."Run Time System" ("Application:Kind")) -> (x = y?=w313:bool)
        n142 = Or(x=w307, y=w313) -> (x .or. y?=w311:bool)
        n143 = Bundle By Name(cluster=w312, "Core.Current VI Reference"=w310, "Core.Close Panel on Exit?"=w311) -> (w317:T12)
        n144 = call <vilib>:"Add State(s) to Queue__JKI_lib_State_Machine.vi"("State(s) in (\"\")"=w319) -> ("States Out"=w318:string)  [unwired: 14 in]
      }
      frame "Error Handler" {
        # "Unhandled Error -- Display it"
        # "Handle any errors here.\nYou can also output any states to clean-up after errors occur"
        # "Clear error"
        n145 = call <vilib>:"General Error Handler.vi"("error in (no error)"=w323) -> ()  [unwired: 10 in, 5 out]
        n146 = call <vilib>:"Add State(s) to Queue__JKI_lib_State_Machine.vi"("State(s) in Front (\"\")"="/* Post Error States", "State(s) in (\"\")"=w327) -> ("States Out"=w326:string)  [unwired: 13 in]
      }
      frame "Exit" {
        # "Do not put any code in this frame.\n(No errors that occur here will be handled.)"
        n147 = call <vilib>:"Add State(s) to Queue__JKI_lib_State_Machine.vi"("State(s) in (\"\")"=w334) -> ("States Out"=w333:string)  [unwired: 14 in]
      }
      frame "---------- Data ----------" {
        # "Do not put any code in this frame.\n(It is a separator no-op. You can make a copy of this frame to create a new Data frame)"
        n148 = call <vilib>:"Add State(s) to Queue__JKI_lib_State_Machine.vi"("State(s) in (\"\")"=w340) -> ("States Out"=w339:string)  [unwired: 14 in]
      }
      frame "Data: Initialize" {
        w342 = refnum<queue> refnum  # LoggerWatchDogQueue
        w343 = path ""  # LogFile
        w344 = refnum<vi>[] []  # Toolbar.Advance
        w346 = T13 {"Current VI Reference"=refnum, "Close Panel on Exit?"=FALSE}  # Core
        # "Data names and types of shift register data are defined by this bundle."
        # "Initialize the shift-register data, here.\n(data names are defined by what you wire into the bundle function)"
        n149 = Bundle("Core"=w346, "Toolbar.Advance"=w344, "LoggerWatchDogQueue"=w342, "LogFile"=w343) -> (w348:T12)  [unwired: 1 in]
        n150 = call <vilib>:"Add State(s) to Queue__JKI_lib_State_Machine.vi"("State(s) in (\"\")"=w350) -> ("States Out"=w349:string)  [unwired: 14 in]
      }
      frame "Data: Initialize References" {
      }
      frame "Data: Cleanup" {
        # "Cleanup any data and references, here.\n(this is called automatically, by the Macro: Exit)"
        n151 = Unbundle By Name(w358) -> ("Core.Current VI Reference"=w361:refnum<vi>)
        n152 = Close Reference(reference=w361, error in (no error)=w360) -> (error out=w359:errorcluster)
        n153 = call <vilib>:"Add State(s) to Queue__JKI_lib_State_Machine.vi"("State(s) in (\"\")"=w363) -> ("States Out"=w362:string)  [unwired: 14 in]
      }
      frame "---------- UI ----------" {
        # "Do not put any code in this frame.\n(It is a separator no-op. You can make a copy of this frame to create a new UI frame)"
        n154 = call <vilib>:"Add State(s) to Queue__JKI_lib_State_Machine.vi"("State(s) in (\"\")"=w369) -> ("States Out"=w368:string)  [unwired: 14 in]
      }
      frame "UI: Initialize" {
        # "Initialize the User Interface, here.\n(this is called automatically, by the Macro: Init)"
        n155 = Unbundle By Name(w383) -> ("Toolbar.Advance"=w382:refnum<vi>[])
        n156 = disable-structure shown="Disabled" {
          disable-tunnel: w382 -> [w388 _]
          frame Disabled {
            n157 = for {
              tunnel: w388 -> [w390] mode=indexing
              n158 = property class="Bool"(reference=w390, "Visible"=FALSE) -> ()  [unwired: 1 in, 2 out]
            }
          }
          frame Enabled {
          }
        }
        n159 = local write "Peroid Logs"(TRUE ("Filter Peroid Logs")) -> ()
        n160 = control-ref of="LogInQ"() -> (w376:refnum<vi>)
        n161 = control-ref of="Level"() -> (w377:refnum<vi>)
        n162 = control-ref of="LogInQ change(#/s)"() -> (w378:refnum<vi>)
        n163 = control-ref of="log handling Speed(#/s)"() -> (w379:refnum<vi>)
        n164 = control-ref of="Peroid Logs"() -> (w372:refnum<vi>)
        n165 = control-ref of="Error(#)"() -> (w373:refnum<vi>)
        n166 = control-ref of="Toolbar.History Length(char)"() -> (w371:refnum<vi>)
        n167 = Build Array(w376, w377, w378, w379) -> (w375:refnum<vi>[])
        n168 = Build Array(w371, w372, w373) -> (w374:refnum<vi>[])
        n169 = call "Distribute Controls Evenly.vi"("space(6)"=u32 3, "Controls"=w375) -> ()  [unwired: 9 in, 1 out]
        n170 = call "Distribute Controls Evenly.vi"("Controls"=w374) -> ()  [unwired: 10 in, 1 out]
        n171 = call <vilib>:"Add State(s) to Queue__JKI_lib_State_Machine.vi"("State(s) in (\"\")"=w387) -> ("States Out"=w386:string)  [unwired: 14 in]
      }
      frame "UI: Cursor Set" {
        # "Argument"
        # "Set and Unset Cursor Busy.\n(Usage: \"UI: Cursor Set >> Busy|Idle\")"
        n172 = case shown="\"Idle\", Default" w393 {
          tunnel: w395 -> [w400 w402]
          tunnel: [w399 w401] -> w394
          frame "Idle", Default {
            n173 = call <vilib>:"Unset Busy.vi"("error in (no error)"=w400) -> ("error out"=w399:errorcluster)  [unwired: 10 in]
          }
          frame "Busy" {
            n174 = call <vilib>:"Set Busy.vi"("error in (no error)"=w402) -> ("error out"=w401:errorcluster)  [unwired: 9 in, 1 out]
          }
        }
        n175 = call <vilib>:"Add State(s) to Queue__JKI_lib_State_Machine.vi"("State(s) in (\"\")"=w398) -> ("States Out"=w397:string)  [unwired: 14 in]
      }
      frame "UI: Front Panel State" {
        # "Argument"
        # "Set Front Panel Open or Closed\n(Usage: \"UI: Front Panel State >> Open|Close\")"
        n176 = Unbundle By Name(w407) -> ("Core.Current VI Reference"=w406:refnum<vi>)
        n177 = case shown="\"Minimize\", \"Minimized\"" w405 {
          tunnel: w409 -> [w417 w432 w443 w456 w469]
          tunnel: [w419 w433 w445 w458 w471] -> w408
          tunnel: w406 -> [w418 w430 w444 w457 w470]
          frame "Open", "Standard", Default {
            w412 = T8."Standard" ("State")
            n178 = property class="VI"(reference=w418, error in=w417) -> (reference out=w415:refnum<vi>, error out=w416:errorcluster, "FP.State"=w414:T8)
            n179 = Not Equal?(x=w414, y=w412) -> (x != y?=w413:bool)
            n180 = case shown="True" w413 {
              tunnel: [w423 w425] -> w419
              tunnel: w416 -> [w422 w425]
              tunnel: w415 -> [w421 _]
              tunnel: w412 -> [w420 _]
              frame True {
                n181 = invoke class="VI" method="FP.Open"(reference=w421, error in=w422, "Activate"=TRUE, "State"=w420) -> (error out=w423:errorcluster)  [unwired: 1 in, 4 out]
              }
              frame False {
              }
            }
          }
          frame "Close", "Closed" {
            n182 = property class="VI"(reference=w430, error in=w432) -> (reference out=w429:refnum<vi>, error out=w431:errorcluster, "FP.State"=w427:T8)
            n183 = Not Equal?(x=w427, y=T8."Closed" ("Front Panel Window:State")) -> (x != y?=w426:bool)
            n184 = case shown="True" w426 {
              tunnel: [w434 w437] -> w433
              tunnel: w431 -> [w434 w436]
              tunnel: w429 -> [_ w435]
              frame False {
              }
              frame True {
                n185 = invoke class="VI" method="FP.Close"(reference=w435, error in=w436) -> (error out=w437:errorcluster)  [unwired: 1 in, 2 out]
              }
            }
          }
          frame "Hidden", "Hide" {
            w438 = T8."Hidden" ("State")
            n186 = property class="VI"(reference=w444, error in=w443) -> (reference out=w441:refnum<vi>, error out=w442:errorcluster, "FP.State"=w440:T8)
            n187 = Not Equal?(x=w440, y=w438) -> (x != y?=w439:bool)
            n188 = case shown="True" w439 {
              tunnel: [w449 w450] -> w445
              tunnel: w442 -> [w448 w450]
              tunnel: w441 -> [w447 _]
              tunnel: w438 -> [w446 _]
              frame True {
                n189 = invoke class="VI" method="FP.Open"(reference=w447, error in=w448, "State"=w446) -> (error out=w449:errorcluster)  [unwired: 2 in, 4 out]
              }
              frame False {
              }
            }
          }
          frame "Minimize", "Minimized" {
            w451 = T8."Minimized" ("State")
            n190 = property class="VI"(reference=w457, error in=w456) -> (reference out=w454:refnum<vi>, error out=w455:errorcluster, "FP.State"=w453:T8)
            n191 = Not Equal?(x=w453, y=w451) -> (x != y?=w452:bool)
            n192 = case shown="True" w452 {
              tunnel: [w462 w463] -> w458
              tunnel: w455 -> [w461 w463]
              tunnel: w454 -> [w460 _]
              tunnel: w451 -> [w459 _]
              frame True {
                n193 = invoke class="VI" method="FP.Open"(reference=w460, error in=w461, "State"=w459) -> (error out=w462:errorcluster)  [unwired: 2 in, 4 out]
              }
              frame False {
              }
            }
          }
          frame "Maximize", "Maximized" {
            w464 = T8."Maximized" ("State")
            n194 = property class="VI"(reference=w470, error in=w469) -> (reference out=w467:refnum<vi>, error out=w468:errorcluster, "FP.State"=w466:T8)
            n195 = Not Equal?(x=w466, y=w464) -> (x != y?=w465:bool)
            n196 = case shown="True" w465 {
              tunnel: [w475 w476] -> w471
              tunnel: w468 -> [w474 w476]
              tunnel: w467 -> [w473 _]
              tunnel: w464 -> [w472 _]
              frame True {
                n197 = invoke class="VI" method="FP.Open"(reference=w473, error in=w474, "State"=w472) -> (error out=w475:errorcluster)  [unwired: 2 in, 4 out]
              }
              frame False {
              }
            }
          }
        }
        n198 = call <vilib>:"Add State(s) to Queue__JKI_lib_State_Machine.vi"("State(s) in (\"\")"=w411) -> ("States Out"=w410:string)  [unwired: 14 in]
      }
      frame "UI: Update Toolbar" {
        w485 = i16 2 ("x")
        n199 = control-ref of="Record.Start"() -> (w493:refnum<vi>)
        n200 = control-ref of="Record.Stop"() -> (w492:refnum<vi>)
        n201 = Unbundle By Name(w491) -> ("Core.Current VI Reference"=w482:refnum<vi>, "LogFile"=w479:path, "LoggerWatchDogQueue"=w490:refnum<queue>)
        n202 = Not A Number/Path/Refnum?(number/path/refnum=w490) -> (NaN/Path/Refnum?=w483:bool)
        n203 = Not(x=w483) -> (.not. x?=w484:bool)
        n204 = Boolean To (0,1)(Boolean=w484) -> (0, 1=w489:i16)
        n205 = Boolean To (0,1)(Boolean=w483) -> (0, 1=w488:i16)
        n206 = Multiply(x=w485, y=w488) -> (x*y=w486:i16)
        n207 = Multiply(x=w485, y=w489) -> (x*y=w487:i16)
        n208 = Empty String/Path?(string/path=w479) -> (empty?=w478:bool)
        n209 = property class="Bool"(reference=w493, "DisabledEnum"=w487) -> ()  [unwired: 1 in, 2 out]
        n210 = property class="Bool"(reference=w492, "DisabledEnum"=w486) -> ()  [unwired: 1 in, 2 out]
        n211 = case shown="True" w478 {
          tunnel: "Running Log Viewer (CSM)" ("Front Panel Window:Title") -> [w501 w502]
          tunnel: [w500 w502] -> w480
          tunnel: w479 -> [w497 _]
          frame False {
            n212 = Path To String(path=w497) -> (string=w498:string)
            n213 = Concatenate Strings(w501, " - " ("string"), w498) -> (w500:string)
          }
          frame True {
          }
        }
        n214 = property class="VI"(reference=w482, "Front Panel.Title"=w480) -> ()  [unwired: 1 in, 2 out]
      }
      frame "UI: Resize Tab Content" {
        n215 = control-ref of="Tab"() -> (w510:refnum<vi>)
        n216 = invoke class="TabCtl (strict)" method="FitControlToPane"(reference=w510) -> (reference out=w507:refnum<vi>, error out=w505:errorcluster)  [unwired: 2 in, 1 out]
        n217 = control-ref of="Global Filters"() -> (w503:refnum<vi>)
        n218 = control-ref of="Error History"() -> (w509:refnum<vi>)
        n219 = control-ref of="State History"() -> (w508:refnum<vi>)
        n220 = control-ref of="Userlog History"() -> (w504:refnum<vi>)
        n221 = Build Array(w504, w509, w508, w503) -> (w506:refnum<vi>[])
        n222 = for {
          tunnel: w507 -> [w518]
          tunnel: w506 -> [w517] mode=indexing
          tunnel: w505 -> [w516]
          n223 = call "Fit Control to Tab.vi"("Control"=w517, "error in (no error)"=w516, "TabRef"=w518) -> ()  [unwired: 4 in, 3 out]
        }
      }
      frame "---------- Macro ----------" {
        # "Do not put any code in this frame.\n(It is a separator no-op. You can make a copy of this frame to create a new Macro frame)"
        n224 = call <vilib>:"Add State(s) to Queue__JKI_lib_State_Machine.vi"("State(s) in (\"\")"=w524) -> ("States Out"=w523:string)  [unwired: 14 in]
      }
      frame "Macro: Initialize" {
        w527 = "Data: Initialize\nData: Initialize References\nInitialize Core Data\nUI: Initialize\nUI: Front Panel State >> Open\nUI: Resize Tab Content\nUI: Update Toolbar"  # Data: Initialize Data: Initialize References Initialize Core Data UI: Initialize UI: Front Panel State >> Open UI: Resize Tab Content UI: Update Toolbar
        # "Initialization Macro\n(This is called once, when the VI starts)"
        n225 = call <vilib>:"Add State(s) to Queue__JKI_lib_State_Machine.vi"("State(s) in Front (\"\")"=w527, "State(s) in (\"\")"=w531) -> ("States Out"=w530:string)  [unwired: 13 in]
      }
      frame "Macro: Exit" {
        (unwired) ""
        # "Exit Macro\n(This is called once, when the VI exits)"
        n226 = Unbundle By Name(w536) -> ()  [unwired: 1 out]
        n227 = call <vilib>:"Add State(s) to Queue__JKI_lib_State_Machine.vi"("State(s) at Back (\"\")"="Data: Cleanup\nExit") -> ("States Out"=w534:string)  [unwired: 14 in]
        n228 = call <vilib>:"Add State(s) to Queue__JKI_lib_State_Machine.vi"("State(s) in Front (\"\")"=w534, "State(s) in (\"\")"=w539) -> ("States Out"=w538:string)  [unwired: 13 in]
      }
    }
  }
  n229 = disable-structure shown="Disabled" {
    frame Disabled {
      n230 = call "CSM - Module VI Reference.vi"("Response Timeout (-2 Using Global Settings)"=1000 ("Response Timeout(5000 ms)"), "error in (no error)"=errorcluster {"status"=FALSE, "code"=0, "source"=""}, "CSM Name"="") -> ("error out"=w546:errorcluster, "CSM Module VIRef"=w545:refnum<vi>)  [unwired: 7 in]
      n231 = invoke on="Invoke Node" class="VI" method="FP.Open"(reference=w545, error in=w546, "Activate"=TRUE ("Activate?")) -> (error out=w544:errorcluster)  [unwired: 2 in, 4 out]
      n232 = call <vilib>:"Simple Error Handler.vi"("error in (no error)"=w544) -> ()  [unwired: 4 in, 5 out]
    }
    frame Enabled {
    }
  }
  n233 = flat-sequence {
    tunnel: [w548] -> w7
    tunnel: w6 -> [w548]
    frame #0 {
      n234 = local write "Stop"(TRUE ("Stop")) -> ()
    }
  }
  n235 = call "CSM - Destroy Global Log Queue.vi"("Error In"=w16, "Global Log Queue"=w14) -> ("error out"=w8:errorcluster)  [unwired: 9 in]
  n236 = control-ref of="Current VI Reference"() -> (w4:refnum<vi>)
  n237 = Merge Errors(w7, w8) -> (w2:errorcluster)
  n238 = call "Close FP if in LabVIEW Dir.vi"("VI Refnum"=w4, "Error in"=w2) -> ("Error out"=w5:errorcluster)  [unwired: 9 in]
  n239 = call <vilib>:"Clear Errors.vi"("error in (no error)"=w5) -> ()  [unwired: 5 in, 2 out]
